vi "remove Line Feed Constant.vi"(11 "Input String":string) -> (3 "Line Feed Removed String":string)   [LabVIEW 2023, in "Spectrum Analyzer.lvlib"]
uses:
  Spectrum Analyzer.lvlib
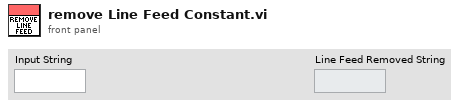
[diagram p1: front panel]
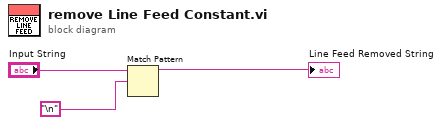
[diagram p0: block diagram]
diagram:
  n1 = Match Pattern(string="Input String", regular expression="\n") -> (before substring=→"Line Feed Removed String":string)  [unwired: 1 in, 3 out]
